vi "Execute.vi"(8 "error in":errorcluster, 9 "Consumer Queues in":T1, 10 "DAC Process Command in":refnum<class "Save DAC Configuration.lvclass">, 11 "DAC Process Data in":T2) -> (0 "error out":errorcluster, 1 "Consumer Queues out":T1, 2 "Stop?":bool, 3 "DAC Process Data out":T2)   [LabVIEW 2019, in "DAC Process.lvlib" / "Save DAC Configuration.lvclass"]
uses:
  Save DAC Configuration.lvclass
  C:/Users/wg/Documents/LV_Projects/test-stand/App/DAC Process/Generic DAC Command/Generic DAC Process Command.lvclass
  DAC Process Data.ctl
  Generic Test Stand/Generic Test Stand.lvclass
  TS Framework/ExeLogging/DAC Logger/DAC Logger.lvclass
  DAC State.ctl
  TS Framework/Consumer Queues.ctl
  UI Process/Generic UI Command/Generic UI Process Command.lvclass
  Generic DAC Command/Generic DAC Process Command.lvclass
  Trig Process/Generic Trig Command/Generic Trig Process Command.lvclass
  UI Process/Update UI Status/Update UI Status.lvclass
  Generic Test Stand/Generic Test Stand.lvclass/Generic Test Stand.ctl
  Generic DAC Command/Generic DAC Process Command.lvclass/Generic DAC Process Command.ctl
  UI Process/Update UI Status/Update UI Status.lvclass/Update UI Status.ctl
  C:/Users/wg/Documents/LV_Projects/test-stand/App/Generic Command/Generic Command.lvclass
  DAC Process.lvlib
  TS Framework/TS Framework.lvlib
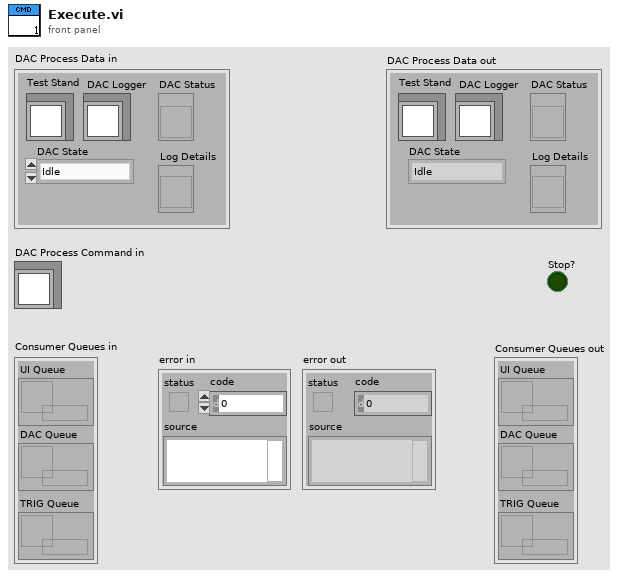
[diagram p1: front panel]
types:
  T1 = typedef "TS Framework.lvlib/Consumer Queues.ctl" = cluster{"UI Queue":refnum<queue>, "DAC Queue":refnum<queue>, "TRIG Queue":refnum<queue>}
  T2 = typedef "DAC Process.lvlib/DAC Process Data.ctl" = cluster{"Test Stand":refnum<class "Generic Test Stand.lvclass">, " DAC Logger":refnum<class "DAC Logger.lvclass">, "DAC State":T3, "DAC Status":refnum<vi>, "Log Details":refnum<vi>}
  T3 = typedef "DAC Process.lvlib/DAC State.ctl" = enum16{"Idle", "Acquiring"}
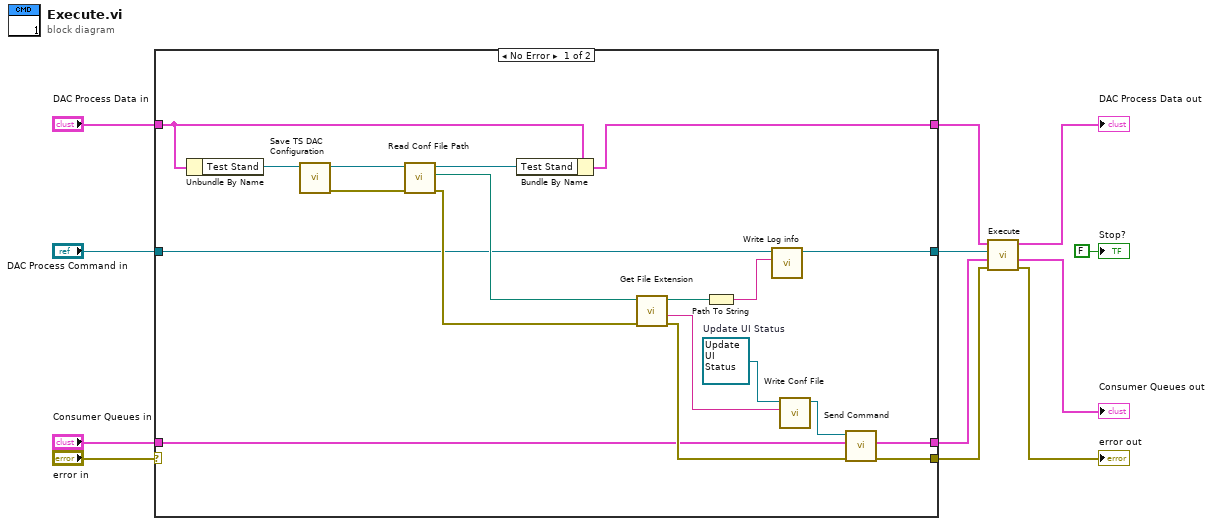
[diagram p0: block diagram]
diagram:
  n1 = case shown="No Error" "error in" {
    selector: "error in" -> [_ w35]
    tunnel: [w26 w35] -> w7
    tunnel: "DAC Process Data in" -> [w30 w34]
    tunnel: [w25 w34] -> w5
    tunnel: "Consumer Queues in" -> [w19 w32]
    tunnel: [w18 w32] -> w3
    tunnel: [w16 w33] -> w2
    tunnel: "DAC Process Command in" -> [w17 w33]
    frame No Error {
      w28 = refnum<class "Update UI Status.lvclass"> refnum  # Update UI Status
      n2 = Unbundle By Name(w30) -> ("Test Stand"=w31:refnum<class "Generic Test Stand.lvclass">)
      n3 = call-dynamic "Save TS DAC Configuration.vi"("Generic Test Stand in"=w31) -> ("error out"=w21:errorcluster, "Generic Test Stand out"=w24:refnum<class "Generic Test Stand.lvclass">)  [unwired: 9 in]
      n4 = call "Read Conf File Path.vi"("error in"=w21, "Generic Test Stand in"=w24) -> ("error out"=w20:errorcluster, "Conf File Path"=w22:path, "Generic Test Stand out"=w23:refnum<class "Generic Test Stand.lvclass">)  [unwired: 7 in]
      n5 = Bundle By Name(cluster=w30, "Test Stand"=w23) -> (w25:T2)
      n6 = call <vilib>:"Get File Extension.vi"("error in (no error)"=w20, "file"=w22) -> ("error out"=w27:errorcluster, "filename without extension"=w15:string, "dup file"=w14:path)  [unwired: 5 in, 2 out]
      n7 = Path To String(path=w14) -> (string=w13:string)
      n8 = call "Write Log info.vi"("Log info"=w13, "Generic DAC Process Command in"=w17) -> ("Generic DAC Process Command out"=w16:refnum<class "Save DAC Configuration.lvclass">)  [unwired: 9 in]
      n9 = call "Write Conf File.vi"("Conf File"=w15, "Update UI Status in"=w28) -> ("Update UI Status out"=w29:refnum<class "Update UI Status.lvclass">)  [unwired: 9 in]
      n10 = call-dynamic "Send Command.vi"("error in (no error)"=w27, "Consumer Queues in"=w19, "UI Process Command in"=w29) -> ("error out"=w26:errorcluster, "Consumer Queues out"=w18:T1)  [unwired: 7 in]
    }
    frame Error {
    }
  }
  n11 = call-parent "Execute.vi"("error in"=w7, "Consumer Queues in"=w3, "DAC Process Command in"=w2, "DAC Process Data in"=w5) -> ("error out"=→"error out":errorcluster, "Consumer Queues out"=→"Consumer Queues out":T1, "DAC Process Data out"=→"DAC Process Data out":T2)  [unwired: 4 in, 1 out]
  "Stop?" <- FALSE ("Stop?")
